vi "CSE routine - Get Top-level Instance Refnum.vi"(8 "error in":errorcluster, 10 "Level (0:Topmost)":i32, 11 "CSE Refnum":T1) -> (0 "error out":errorcluster, 1 "Current Instance Level":i32, 2 "Top-level CSE Instance Refnum":T1, 3 "dup CSE Refnum":T1)   [LabVIEW 2021]
doc: "::: CalcExpress Toolkit :::\nCopyright (c) 2000-2026 Konstantin Shifershteyn. All rights reserved."
uses:
  CSE Instance RefNum.ctl
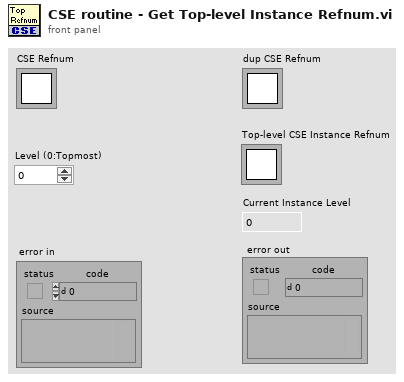
[diagram p1: front panel]
types:
  T1 = typedef "CSE Instance RefNum.ctl" = refnum<k1>
  T2 = cluster{"level":i32, "Caller CSE RefNum":T1, "Callee CSE RefNum":T1}
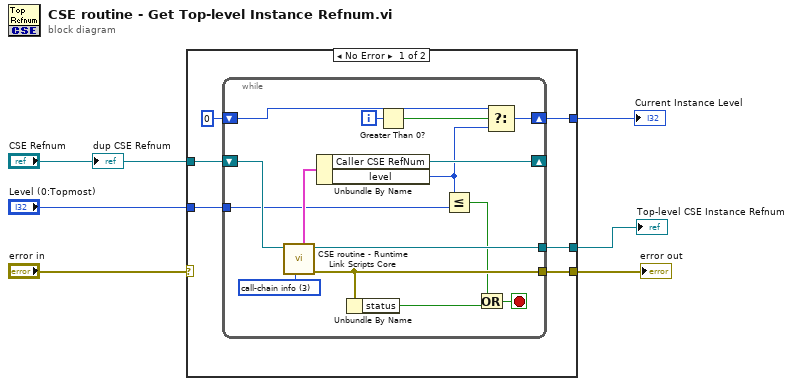
[diagram p0: block diagram]
diagram:
  n1 = case shown="No Error" "error in" {
    selector: "error in" -> [_ w28]
    tunnel: [w12 _] -> w6
    tunnel: [w11 w28] -> w5
    tunnel: "CSE Refnum" -> [w10 _]
    tunnel: "Level (0:Topmost)" -> [w9 _]
    tunnel: [w8 _] -> w1
    frame No Error {
      n2 = while {
        shift-right: [w24] -> _
        shift-left: w10 -> [w25]
        tunnel: [w23] -> w12
        tunnel: [w20] -> w11
        tunnel: w9 -> [w19]
        shift-right: [w14] -> w8
        shift-left: 0 ("level") -> [w13]
        i -> [w17]
        stop <- w22 stop-if-true
        w27 = 3 items=["save vi path", "link to caller", "delink of caller", "call-chain info"] ("action")
        n3 = call "CSE routine - Runtime Link Scripts Core.vi"("action"=w27, "CSE RefNum"=w25) -> ("error out"=w20:errorcluster, "dup CSE RefNum"=w23:T1, "call-chain info"=w26:T2)  [unwired: 4 in, 3 out]
        n4 = Unbundle By Name(w26) -> ("Caller CSE RefNum"=w24:T1, "level"=w15:i32)
        n5 = Unbundle By Name(w20) -> ("status"=w21:bool)
        n6 = Greater Than 0?(x=w17) -> (x > 0?=w16:bool)
        n7 = Less Or Equal?(x=w15, y=w19) -> (x <= y?=w18:bool)
        n8 = Or(x=w18, y=w21) -> (x .or. y?=w22:bool)
        n9 = Select(t=w13, s=w16, f=w15) -> (s? t:f=w14:i32)
      }
    }
    frame Error {
    }
  }
  "error out" <- w5
  "Top-level CSE Instance Refnum" <- w6
  "Current Instance Level" <- w1
  "dup CSE Refnum" <- "CSE Refnum"
